vi "xlsx to Cluster.vi"(7 "Excel._SheetName":string="Sheet1", 8 "Error (in)":errorcluster, 11 "file path (dialog if empty)":path) -> (0 "Error (out)":errorcluster, 2 "All Octal?":bool, 3 "Parameter Array":T1[](array[typedef]))   [LabVIEW 2023]
uses:
  Controls/Database_Array.ctl
  Controls/Encoding.ctl
  <vilib>/Utility/error.llb/Trim Whitespace One-Sided.vi
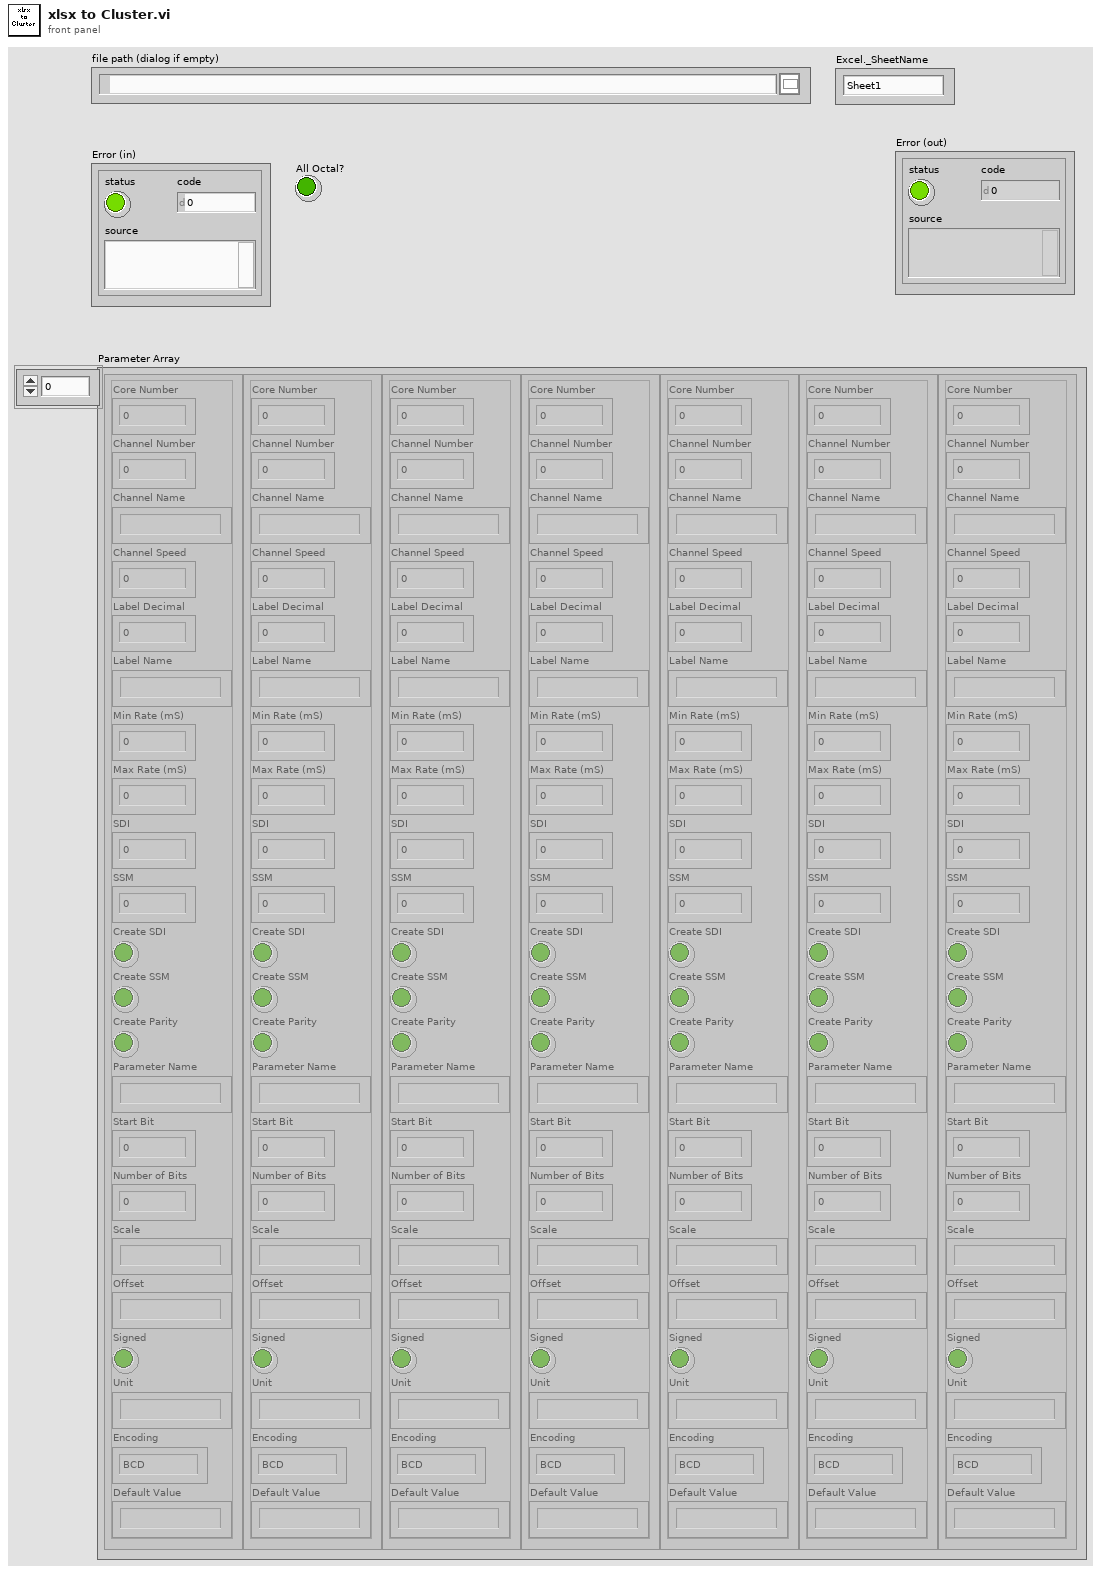
[diagram p1: front panel]
types:
  T1 = typedef "Database_Array.ctl" = cluster{"Core Number":i32, "Channel Number":i32, "Channel Name":string, "Channel Speed":i32, "Label Decimal":u32, "Label Name":string, "Min Rate (mS)":i32, "Max Rate (mS)":i32, "SDI":i32, "SSM":i32, "Create SDI":bool, "Create SSM":bool, "Create Parity":bool, "Parameter Name":string, "Start Bit":i32, "Number of Bits":i32, "Scale":string, "Offset":string, "Signed":bool, "Unit":string, "Encoding":T2, "Default Value":string}
  T2 = typedef "Encoding.ctl" = enum16{"BCD", "BNR", "Discrete"}
  T3 = enum16{"Channel Error", "Label Error", "Octal Error"}
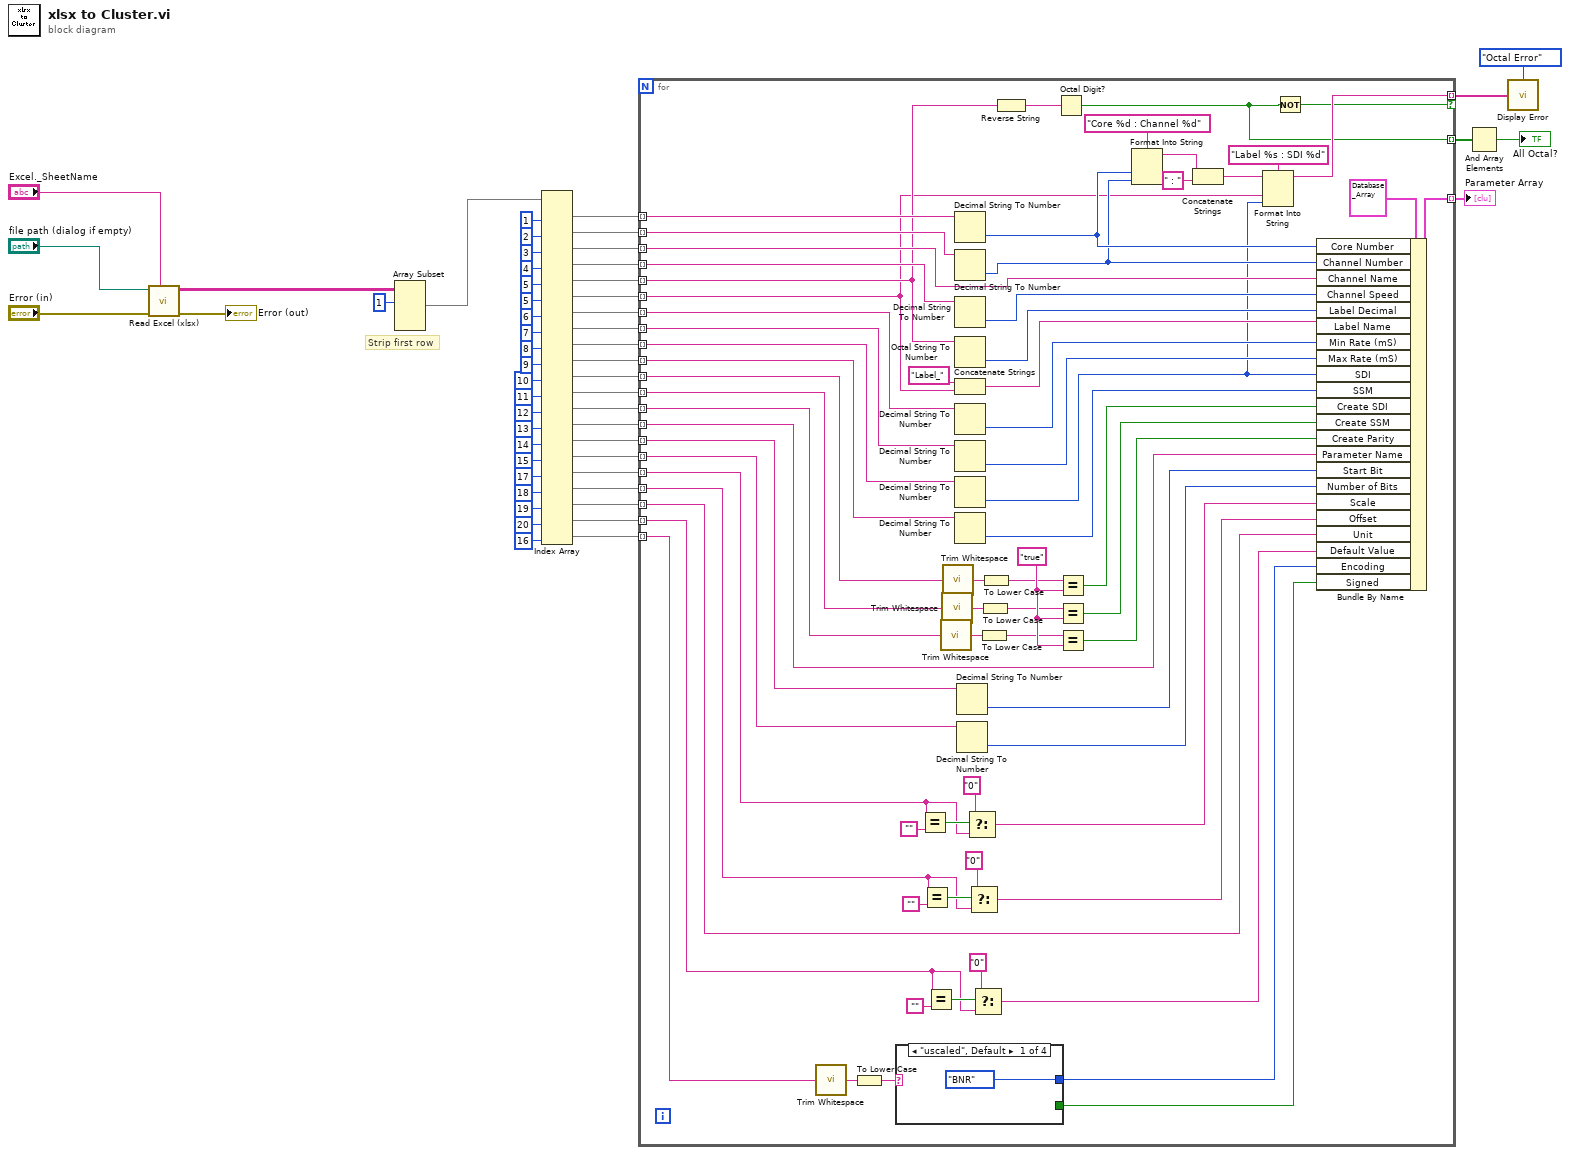
[diagram p0: block diagram]
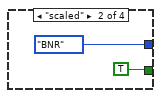
[diagram p2: hidden frame]
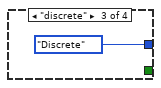
[diagram p3: hidden frame]
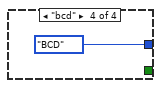
[diagram p4: hidden frame]
diagram:
  # "Strip first row"
  n1 = call "Read Excel (xlsx).vi"("Excel._SheetName"="Excel._SheetName", "error in (no error)"="Error (in)", "File Path Control"="file path (dialog if empty)") -> ("error out"=→"Error (out)":errorcluster, "data"=w52:string[][])  [unwired: 7 in]
  n2 = Array Subset(array=w52, index (row)=1 ("index")) -> (w30:string[][])  [unwired: 3 in]
  n3 = Index Array(array=w30, index (col) #1=1 ("disabled index (col)"), index (col) #2=2 ("disabled index (col)"), index (col) #3=3 ("index (col)"), index (col) #4=4 ("index (col)"), index (col) #5=5 ("index (col)"), index (col) #6=5 ("index (col)"), index (col) #7=6 ("index (col)"), index (col) #8=7 ("index (col)"), index (col) #9=8 ("index (col)"), index (col) #10=9 ("index (col)"), index (col) #11=10 ("index (col)"), index (col) #12=11 ("index (col)"), index (col) #13=12 ("index (col)"), index (col) #14=13 ("index (col)"), index (col) #15=14 ("index (col)"), index (col) #16=15 ("index (col)"), index (col) #17=17 ("index (col)"), index (col) #18=18 ("index (col)"), index (col) #19=19 ("index (col)"), index (col) #20=20 ("index (col)"), index (col) #21=16 ("index (col)")) -> (element #1=w31:string[], element #2=w29:string[], element #3=w28:string[], element #4=w27:string[], element #5=w26:string[], element #6=w25:string[], element #7=w24:string[], element #8=w23:string[], element #9=w22:string[], element #10=w21:string[], element #11=w20:string[], element #12=w19:string[], element #13=w18:string[], element #14=w17:string[], element #15=w16:string[], element #16=w15:string[], element #17=w14:string[], element #18=w13:string[], element #19=w12:string[], element #20=w11:string[], element #21=w10:string[])  [unwired: 21 in]
  n4 = for {
    tunnel: [w123] -> w48 mode=indexing
    tunnel: w31 -> [w122] mode=indexing
    tunnel: w29 -> [w121] mode=indexing
    tunnel: w28 -> [w118] mode=indexing
    tunnel: w27 -> [w120] mode=indexing
    tunnel: w26 -> [w68] mode=indexing
    tunnel: w25 -> [w55] mode=indexing
    tunnel: w24 -> [w117] mode=indexing
    tunnel: w23 -> [w116] mode=indexing
    tunnel: w22 -> [w115] mode=indexing
    tunnel: w21 -> [w114] mode=indexing
    tunnel: w20 -> [w102] mode=indexing
    tunnel: w19 -> [w101] mode=indexing
    tunnel: w18 -> [w99] mode=indexing
    tunnel: w17 -> [w97] mode=indexing
    tunnel: w16 -> [w96] mode=indexing
    tunnel: w15 -> [w95] mode=indexing
    tunnel: w14 -> [w86] mode=indexing
    tunnel: w13 -> [w83] mode=indexing
    tunnel: w12 -> [w82] mode=indexing
    tunnel: w11 -> [w77] mode=indexing
    tunnel: w10 -> [w74] mode=indexing
    tunnel: [w58] -> w3 mode=indexing if=w57
    tunnel: [w56] -> w2 mode=indexing
    w109 = "true"
    n5 = call <vilib>:"Trim Whitespace.vi"("string"=w74) -> ("trimmed string"=w76:string)  [unwired: 1 in]
    n6 = To Lower Case(string=w76) -> (all lower case string=w75:string)
    n7 = case shown="\"uscaled\", Default" w75 {
      tunnel: [Encoding."BNR" ("Enum") Encoding."BNR" ("Enum") Encoding."Discrete" ("Enum") Encoding."BCD" ("Enum")] -> w73
      tunnel: [_ TRUE _ _] -> w72
      frame "uscaled", Default {
      }
      frame "scaled" {
      }
      frame "discrete" {
      }
      frame "bcd" {
      }
    }
    n8 = Equal?(x=w86, y="") -> (x = y?=w91:bool)
    n9 = Equal?(x=w83, y="") -> (x = y?=w88:bool)
    n10 = Equal?(x=w77, y="") -> (x = y?=w80:bool)
    n11 = call <vilib>:"Trim Whitespace.vi"("string"=w99) -> ("trimmed string"=w106:string)  [unwired: 1 in]
    n12 = call <vilib>:"Trim Whitespace.vi"("string"=w101) -> ("trimmed string"=w105:string)  [unwired: 1 in]
    n13 = call <vilib>:"Trim Whitespace.vi"("string"=w102) -> ("trimmed string"=w104:string)  [unwired: 1 in]
    n14 = Decimal String To Number(string=w122) -> (number=w66:i32)  [unwired: 2 in, 1 out]
    n15 = Decimal String To Number(string=w121) -> (number=w65:i32)  [unwired: 2 in, 1 out]
    n16 = Decimal String To Number(string=w120) -> (number=w119:i32)  [unwired: 2 in, 1 out]
    n17 = Octal String To Number(4:w68) -> (0:w70:u32)  [unwired: 2 in, 1 out]
    n18 = Concatenate Strings("Label_" ("String"), w55) -> (w60:string)
    n19 = Decimal String To Number(string=w117) -> (number=w113:i32)  [unwired: 2 in, 1 out]
    n20 = Decimal String To Number(string=w116) -> (number=w112:i32)  [unwired: 2 in, 1 out]
    n21 = Decimal String To Number(string=w115) -> (number=w59:i32)  [unwired: 2 in, 1 out]
    n22 = Decimal String To Number(string=w114) -> (number=w111:i32)  [unwired: 2 in, 1 out]
    n23 = Decimal String To Number(string=w96) -> (number=w94:i32)  [unwired: 2 in, 1 out]
    n24 = Decimal String To Number(string=w95) -> (number=w93:i32)  [unwired: 2 in, 1 out]
    n25 = Select(t="0", s=w91, f=w86) -> (s? t:f=w85:string)
    n26 = Select(t="0", s=w88, f=w83) -> (s? t:f=w84:string)
    n27 = Select(t="0", s=w80, f=w77) -> (s? t:f=w78:string)
    n28 = To Lower Case(string=w106) -> (all lower case string=w98:string)
    n29 = To Lower Case(string=w105) -> (all lower case string=w100:string)
    n30 = To Lower Case(string=w104) -> (all lower case string=w103:string)
    n31 = Reverse String(1:w68) -> (0:w69:string)
    n32 = Octal Digit?(1:w69) -> (0:w56:bool)
    n33 = Equal?(x=w103, y=w109) -> (x = y?=w110:bool)
    n34 = Equal?(x=w100, y=w109) -> (x = y?=w108:bool)
    n35 = Equal?(x=w98, y=w109) -> (x = y?=w107:bool)
    n36 = Format Into String(format string="Core %d : Channel %d", w66, w65) -> (resulting string=w62:string)  [unwired: 2 in, 1 out]
    n37 = Concatenate Strings(w62, " : " ("string")) -> (w61:string)
    n38 = Format Into String(format string="Label %s : SDI %d", initial string=w61, w55, w59) -> (resulting string=w58:string)  [unwired: 1 in, 1 out]
    n39 = Not(x=w56) -> (.not. x?=w57:bool)
    n40 = Bundle By Name(cluster=T1 {"Core Number"=0, "Channel Number"=0, "Channel Name"="", "Channel Speed"=0, "Label Decimal"=0, "Label Name"="", "Min Rate (mS)"=0, "Max Rate (mS)"=0, "SDI"=0, "SSM"=0, "Create SDI"=FALSE, "Create SSM"=FALSE, "Create Parity"=FALSE, "Parameter Name"="", "Start Bit"=0, "Number of Bits"=0, "Scale"="", "Offset"="", "Signed"=FALSE, "Unit"="", "Encoding"=enum."BCD", "Default Value"=""} ("Array"), "Core Number"=w66, "Channel Number"=w65, "Channel Name"=w118, "Channel Speed"=w119, "Label Decimal"=w70, "Label Name"=w60, "Min Rate (mS)"=w113, "Max Rate (mS)"=w112, "SDI"=w59, "SSM"=w111, "Create SDI"=w110, "Create SSM"=w108, "Create Parity"=w107, "Parameter Name"=w97, "Start Bit"=w94, "Number of Bits"=w93, "Scale"=w85, "Offset"=w84, "Unit"=w82, "Default Value"=w78, "Encoding"=w73, "Signed"=w72) -> (w123:T1)
  }
  "Parameter Array" <- w48
  n41 = And Array Elements(Boolean array=w2) -> (logical AND=→"All Octal?":bool)
  n42 = call "Display Error.vi"("Error Type"=T3."Octal Error", "Errors"=w3) -> ()  [unwired: 14 in]
